vi "setting.vi"(7 "Level":i32, 10 "型号":string, 11 "型号表":string[](array[string])) -> (2 "型号out":string, 3 "型号表 out":string[](array[string]))   [LabVIEW 2025]
uses:
  global.vi
  <vilib>/Utility/config.llb/Read Key (String).vi
  <vilib>/Utility/config.llb/Write Key (String).vi
  <vilib>/Utility/config.llb/NI_LVConfig.lvlib
panel:
  in  "修改密码":bool caption="ChangePassword"
  in  "Tab":T1(tab)
  in  "CurrentType":enum16{"RMS均方根值", "AVG平均值"}(ring) caption="RMS/AVG Type"
  in  "最大电流":bool caption="Current Enabled"
  in  "平均电流":bool caption="RMS/AVG Enabled"
  in  "最大电流下限":dbl caption="Min Current" format="%#.2f"
  in  "平均电流下限":dbl caption="Min RMS/AVG" format="%#.2f"
  in  "平均电流上限":dbl caption="Max RMS/AVG" format="%#.2f"
  in  "最大电流上限":dbl caption="Max Current" format="%#.2f"
  in  "能量":bool caption="Power Enabled"
  in  "打钉时间":bool caption="Time Enabled"
  in  "能量下限":dbl caption="Min Power" format="%#.2f"
  in  "能量上限":dbl caption="Max Power" format="%#.2f"
  in  "时间下限":dbl caption="Min Time" format="%#.2f"
  in  "时间上限":dbl caption="Max Time" format="%#.2f"
  in  "检查数":dbl=20.0 caption="Check Stop Point"
  in  "PLCPort":string(combo) caption="PLC Port"
  in  "Language":string(combo)
  in  "最大补偿":dbl caption="Max Current  offset" format="%#.2f"
  in  "平均补偿":dbl caption="RMS/AVG Current offset" format="%#.2f"
  in  "能量补偿":dbl caption="Power offset" format="%#.2f"
  in  "时间补偿":dbl caption="Time offset" format="%#.2f"
  in  "单发打钉次数":u32=1 caption="Singe Times" min=1 max=20 step=1
  in  "连发打钉次数":u32=1 caption="Repeating Times" max=10 step=1
  in  "触发值":dbl caption="Trigger Level" format="%#.2f"
  in  "停止值":dbl caption="Stop Level" format="%#.2f"
  in  "倍数":dbl format="%#.2f"
  in  "HighVoltageAlarm":sgl=1.0 caption="High Voltage Alarm" min=1 max=50 step=0.5 format="%.2f"
  in  "LowVoltageAlarm":dbl=1.0 caption="Low Voltage Alarm" min=0.0 max=20.0 step=0.5 format="%.2f"
  in  "Modbus":string(combo)
  in  "另存为":bool caption="As Save"
  in  "退出":bool caption="Exit"
  in  "Save":bool
  # "A"
  # "A"
  # "A"
  # "A"
  # "ms"
  # "ms"
  # "A"
  # "A"
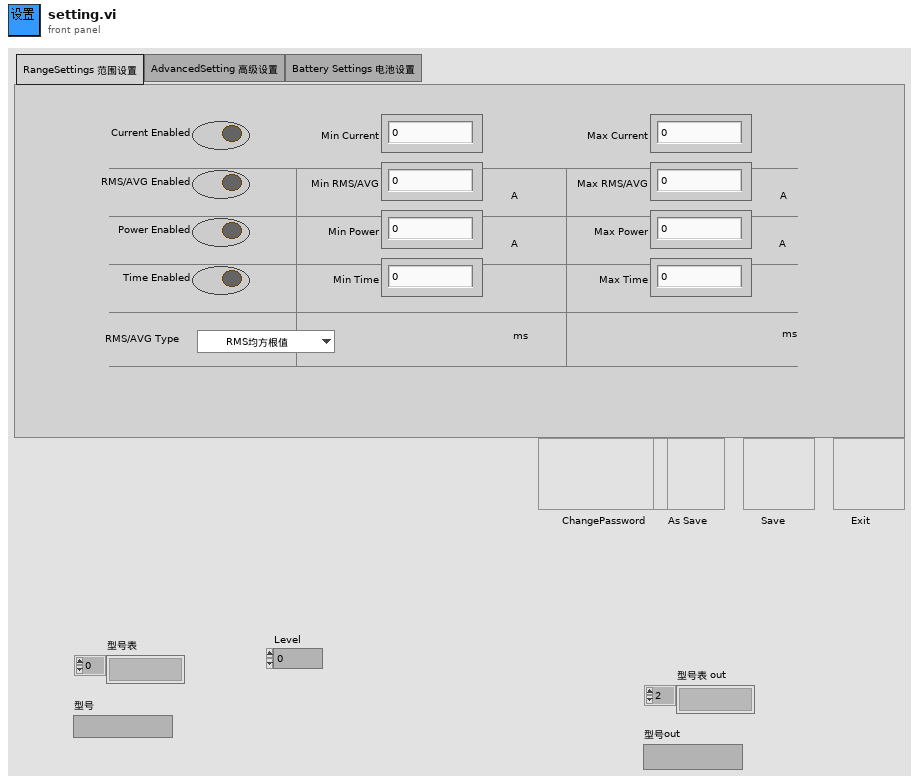
[diagram p1: front panel]
types:
  T1 = enum32{"RangeSettings 范围设置", "AdvancedSetting 高级设置", "Battery Settings 电池设置"}
  T2 = cluster{"Name":string, "Type":string, "DefVal":string}[]
  T3 = typedef "NI_LVConfig.lvlib/Config Data RefNum.ctl" = refnum<k1>
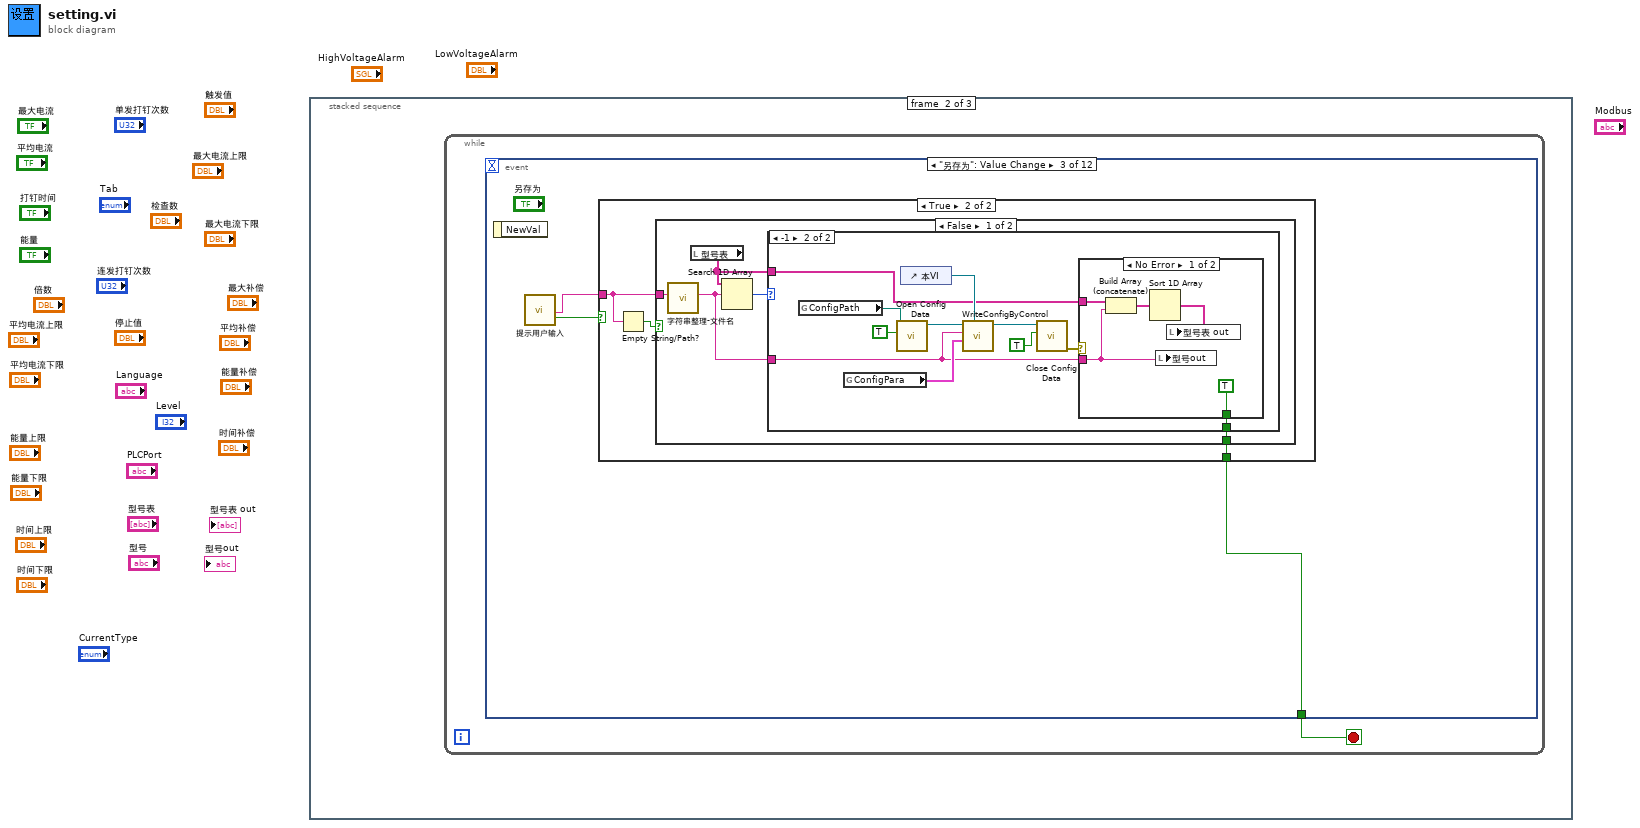
[diagram p0: block diagram]
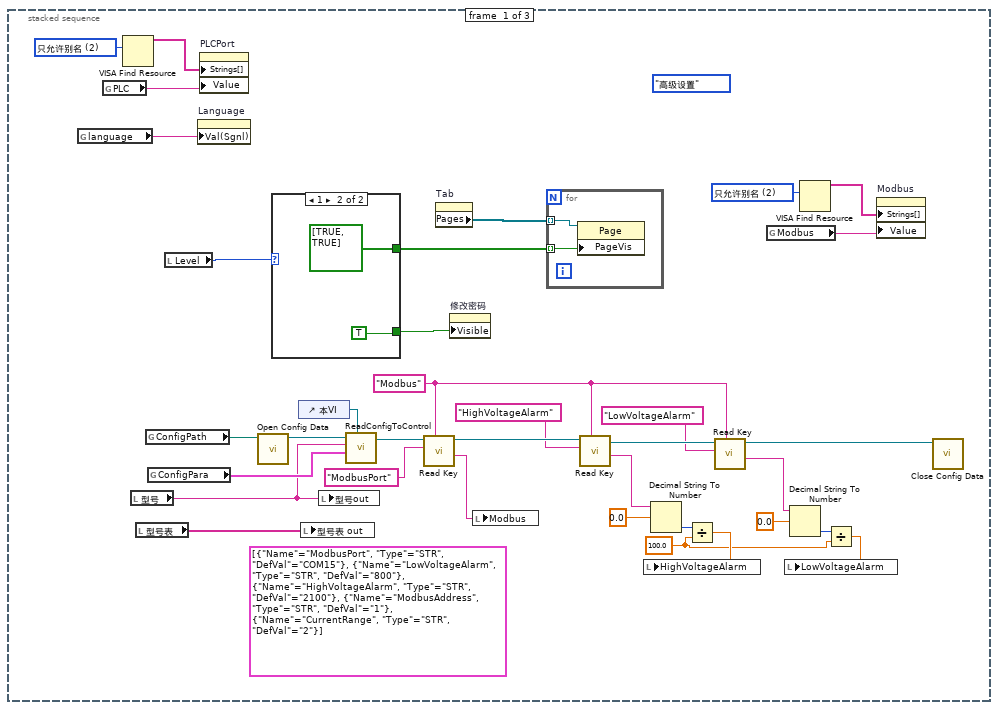
[diagram p2: hidden frame]
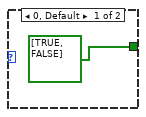
[diagram p3: hidden frame]
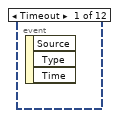
[diagram p4: hidden frame]
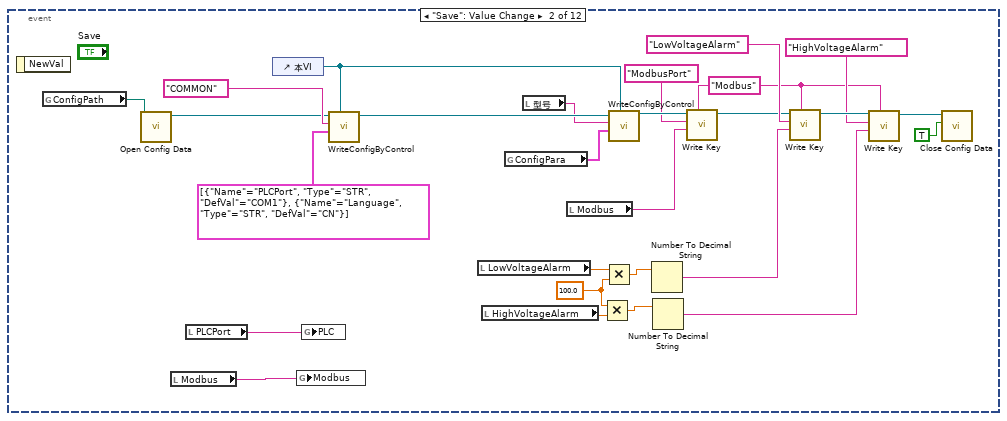
[diagram p5: hidden frame]
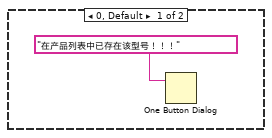
[diagram p7: hidden frame]
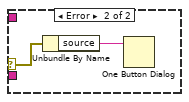
[diagram p8: hidden frame]
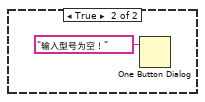
[diagram p9: hidden frame]
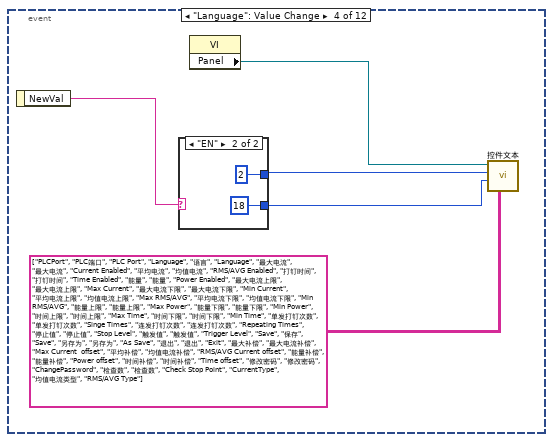
[diagram p10: hidden frame]
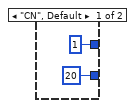
[diagram p11: hidden frame]
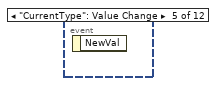
[diagram p12: hidden frame]
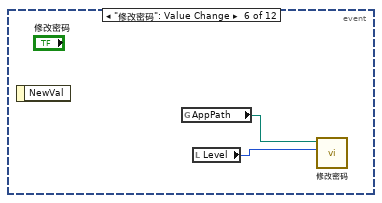
[diagram p13: hidden frame]
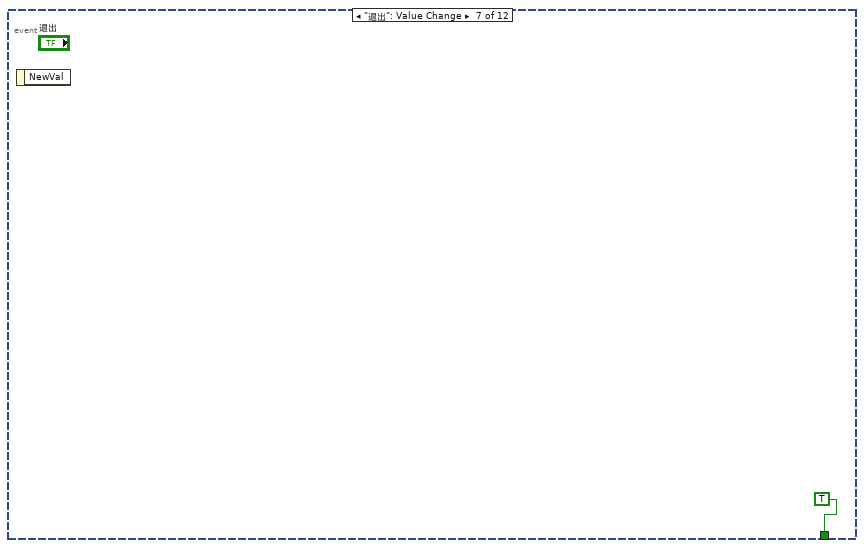
[diagram p14: hidden frame]
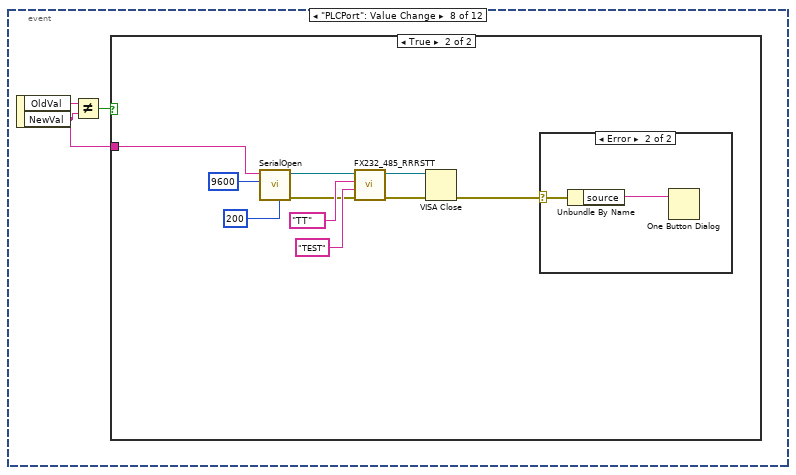
[diagram p15: hidden frame]
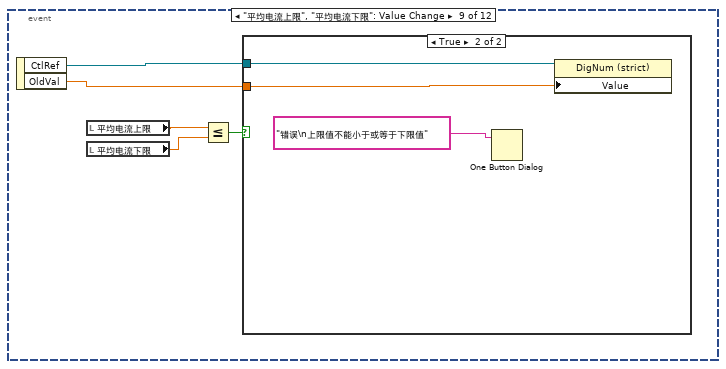
[diagram p18: hidden frame]
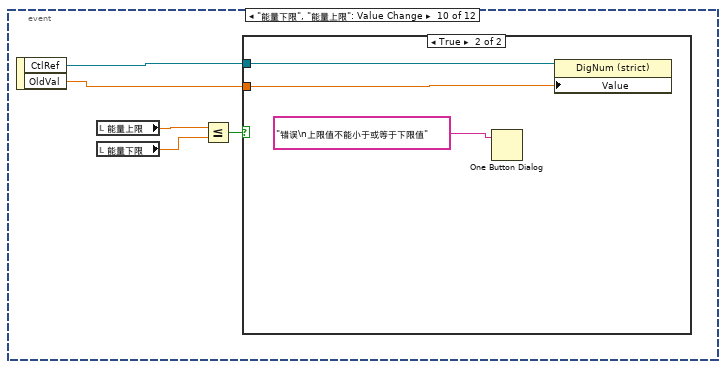
[diagram p20: hidden frame]
diagram:
  n1 = stacked-sequence {
    frame #0 {
      w1 = 100.0
      (unwired) T2 [{"Name"="ModbusPort", "Type"="STR", "DefVal"="COM15"}, {"Name"="LowVoltageAlarm", "Type"="STR", "DefVal"="800"}, {"Name"="HighVoltageAlarm", "Type"="STR", "DefVal"="2100"}, {"Name"="ModbusAddress", "Type"="STR", "DefVal"="1"}, {"Name"="CurrentRange", "Type"="STR", "DefVal"="2"}] ("ModbusConfig")
      w13 = "Modbus" ("section")
      w22 = u32 2 items=["仅允许规范名称"=0, "只允许别名"=2, "包含匹配别名"=3, "包含所有别名"=4] ("Search Mode")
      (unwired) enum32{"范围设置", "高级设置"}."高级设置" ("Tab")
      w35 = u32 2 items=["仅允许规范名称"=0, "只允许别名"=2, "包含匹配别名"=3, "包含所有别名"=4] ("Search Mode")
      n2 = global read "global.vi" "language"() -> (w33:string)
      n3 = global read "global.vi" "PLC"() -> (w32:string)
      n4 = VISA Find Resource(10:w35) -> (3:w34:string[])  [unwired: 2 in, 2 out]
      n5 = local read "型号"() -> (w28:string)
      n6 = local read "型号表"() -> (w27:string[])
      n7 = global read "global.vi" "ConfigPath"() -> (w31:path)
      n8 = global read "global.vi" "ConfigPara"() -> (w29:T2)
      n9 = local read "Level"() -> (w23:i32)
      n10 = property on="Language" class="CmbBox"("Val(Sgnl)"=w33) -> ()  [unwired: 2 in, 2 out]
      n11 = property on="PLCPort" class="CmbBox"("Strings[]"=w34, "Value"=w32) -> ()  [unwired: 2 in, 2 out]
      n12 = call <vilib>:"Open Config Data.vi"("configuration file path"=w31) -> ("refnum"=w30:T3)  [unwired: 8 in, 2 out]
      n13 = case shown="1" w23 {
        tunnel: [bool[] [TRUE, FALSE] bool[] [TRUE, TRUE]] -> w25
        tunnel: [_ TRUE] -> w24
        frame 0, Default {
        }
        frame 1 {
        }
      }
      n14 = control-ref of="本VI"() -> (w19:refnum<vi>)
      n15 = local write "型号表 out"(w27) -> ()
      n16 = local write "型号out"(w28) -> ()
      n17 = call "ReadConfigToControl.vi"("VI引用句柄"=w19, "ConfigInfo"=w29, "section"=w28, "refnum"=w30) -> ("refnum out"=w18:refnum<k1>)  [unwired: 6 in, 1 out]
      n18 = call-poly <vilib>:"Read Key.vi"("section"=w13, "key"="ModbusPort", "refnum"=w18) -> ("value"=w17:string, "refnum out"=w15:T3)  [unwired: 5 in, 2 out]
      n19 = property on="Tab" class="TabCtl (strict)"() -> ("Pages"=w26:refnum<vi>[])  [unwired: 2 in, 2 out]
      n20 = property on="修改密码" class="Bool"("Visible"=w24) -> ()  [unwired: 2 in, 2 out]
      n21 = local write "Modbus"(w17) -> ()
      n22 = for {
        tunnel: w26 -> [w40] mode=indexing
        tunnel: w25 -> [w39] mode=indexing
        n23 = property class="Page"(reference=w40, "PageVis"=w39) -> ()  [unwired: 1 in, 2 out]
      }
      n24 = call-poly <vilib>:"Read Key.vi"("section"=w13, "key"="HighVoltageAlarm", "refnum"=w15) -> ("value"=w9:string, "refnum out"=w12:T3)  [unwired: 5 in, 2 out]
      n25 = Decimal String To Number(string=w9, offset=0.0) -> (number=w7:i32)  [unwired: 1 in, 1 out]
      n26 = Divide(x=w7, y=w1) -> (x/y=w6:dbl)
      n27 = local write "HighVoltageAlarm"(w6) -> ()
      n28 = call-poly <vilib>:"Read Key.vi"("section"=w13, "key"="LowVoltageAlarm", "refnum"=w12) -> ("value"=w4:string, "refnum out"=w10:T3)  [unwired: 5 in, 2 out]
      n29 = global read "global.vi" "Modbus"() -> (w20:string)
      n30 = Decimal String To Number(string=w4, offset=0.0) -> (number=w5:i32)  [unwired: 1 in, 1 out]
      n31 = VISA Find Resource(10:w22) -> (3:w21:string[])  [unwired: 2 in, 2 out]
      n32 = Divide(x=w5, y=w1) -> (x/y=w2:dbl)
      n33 = local write "LowVoltageAlarm"(w2) -> ()
      n34 = property on="Modbus" class="CmbBox"("Strings[]"=w21, "Value"=w20) -> ()  [unwired: 2 in, 2 out]
      n35 = call <vilib>:"Close Config Data.vi"("refnum"=w10) -> ()  [unwired: 9 in, 2 out]
    }
    frame #1 {
      n36 = while {
        stop <- w41 stop-if-true
        n37 = event shown="[2] \"另存为\": Value Change" {
          selector: _ -> [_ _ _ _ _ _ _ _ _ _ _ _]
          dyn-events: _ -> [_ _ _ _ _ _ _ _ _ _ _ _]
          timeout: _ -> [_ _ _ _ _ _ _ _ _ _ _ _]
          tunnel: [_ _ w69 _ _ _ TRUE _ _ _ _ _] -> w41
          event Timeout {
            n38 = event-data() -> ()  [unwired: 1 in, 3 out]
          }
          event "Save": Value Change {
            w49 = 100.0 ("y")
            w46 = "Modbus" ("section")
            n39 = event-data() -> ()  [unwired: 1 in, 1 out]
            n40 = global read "global.vi" "ConfigPath"() -> (w68:path)
            n41 = call <vilib>:"Open Config Data.vi"("configuration file path"=w68) -> ("refnum"=w62:T3)  [unwired: 8 in, 2 out]
            n42 = local read "Modbus"() -> (w59:string)
            n43 = local read "PLCPort"() -> (w61:string)
            n44 = control-ref of="本VI"() -> (w58:refnum<vi>)
            n45 = global write "global.vi" "Modbus"(w59) -> ()
            n46 = global write "global.vi" "PLC"(w61) -> ()
            n47 = call "WriteConfigByControl.vi"("VI引用句柄"=w58, "ConfigInfo"=T2 [{"Name"="PLCPort", "Type"="STR", "DefVal"="COM1"}, {"Name"="Language", "Type"="STR", "DefVal"="CN"}], "section"="COMMON", "refnum"=w62) -> ("refnum out"=w64:refnum<k1>)  [unwired: 6 in, 1 out]
            n48 = local read "LowVoltageAlarm"() -> (w50:dbl)
            n49 = local read "HighVoltageAlarm"() -> (w48:sgl)
            n50 = global read "global.vi" "ConfigPara"() -> (w66:T2)
            n51 = local read "型号"() -> (w60:string)
            n52 = local read "Modbus"() -> (w42:string)
            n53 = Multiply(x=w49, y=w48) -> (x*y=w47:dbl)
            n54 = Multiply(x=w50, y=w49) -> (x*y=w51:dbl)
            n55 = call "WriteConfigByControl.vi"("VI引用句柄"=w58, "ConfigInfo"=w66, "section"=w60, "refnum"=w64) -> ("refnum out"=w45:refnum<k1>)  [unwired: 6 in, 1 out]
            n56 = Number To Decimal String(number=w51) -> (decimal integer string=w53:string)  [unwired: 1 in]
            n57 = Number To Decimal String(number=w47) -> (decimal integer string=w54:string)  [unwired: 1 in]
            n58 = call-poly <vilib>:"Write Key.vi"("section"=w46, "value"=w42, "key"="ModbusPort", "refnum"=w45) -> ("refnum out"=w44:T3)  [unwired: 5 in, 2 out]
            n59 = call-poly <vilib>:"Write Key.vi"("section"=w46, "value"=w53, "key"="LowVoltageAlarm", "refnum"=w44) -> ("refnum out"=w56:T3)  [unwired: 5 in, 2 out]
            n60 = call-poly <vilib>:"Write Key.vi"("section"=w46, "value"=w54, "key"="HighVoltageAlarm", "refnum"=w56) -> ("refnum out"=w52:T3)  [unwired: 5 in, 2 out]
            n61 = call <vilib>:"Close Config Data.vi"("write file if changed (T)"=TRUE, "refnum"=w52) -> ()  [unwired: 8 in, 2 out]
          }
          event "另存为": Value Change {
            n62 = event-data() -> ()  [unwired: 1 in, 1 out]
            n63 = call "提示用户输入"() -> ("产品型号"=w70:string, "确定"=w71:bool)  [unwired: 17 in, 1 out]
            n64 = case shown="True" w71 {
              tunnel: w70 -> [_ w73]
              tunnel: [_ w74] -> w69
              frame False {
              }
              frame True {
                n65 = Empty String/Path?(string/path=w73) -> (empty?=w72:bool)
                n66 = case shown="False" w72 {
                  tunnel: [w78 _] -> w74
                  tunnel: w73 -> [w76 _]
                  frame False {
                    n67 = call "字符串整理-文件名.vi"("输入字符串"=w76) -> ("结果字符串"=w77:string)  [unwired: 10 in]
                    n68 = local read "型号表"() -> (w75:string[])
                    n69 = Search 1D Array(1D array=w75, element=w77) -> (index of element=w79:i32)  [unwired: 1 in]
                    n70 = case shown="-1" w79 {
                      tunnel: w77 -> [_ w83]
                      tunnel: [_ w82] -> w78
                      tunnel: w75 -> [_ w81]
                      frame 0, Default {
                        n71 = One Button Dialog(message="在产品列表中已存在该型号！！！" ("消息")) -> ()  [unwired: 1 in, 1 out]
                      }
                      frame -1 {
                        n72 = global read "global.vi" "ConfigPath"() -> (w91:path)
                        n73 = global read "global.vi" "ConfigPara"() -> (w88:T2)
                        n74 = call <vilib>:"Open Config Data.vi"("create file if necessary (T)"=TRUE, "configuration file path"=w91) -> ("refnum"=w85:T3)  [unwired: 7 in, 2 out]
                        n75 = control-ref of="本VI"() -> (w86:refnum<vi>)
                        n76 = call "WriteConfigByControl.vi"("VI引用句柄"=w86, "ConfigInfo"=w88, "section"=w83, "refnum"=w85) -> ("refnum out"=w87:refnum<k1>)  [unwired: 6 in, 1 out]
                        n77 = call <vilib>:"Close Config Data.vi"("write file if changed (T)"=TRUE, "refnum"=w87) -> ("error out"=w84:errorcluster)  [unwired: 8 in, 1 out]
                        n78 = case shown="No Error" w84 {
                          selector: w84 -> [_ w98]
                          tunnel: w83 -> [w93 _]
                          tunnel: [TRUE _] -> w82
                          tunnel: w81 -> [w94 _]
                          frame No Error {
                            n79 = Build Array (concatenate)(w94, w93) -> (w92:string[])
                            n80 = Sort 1D Array(array=w92) -> (sorted array=w95:string[])
                            n81 = local write "型号out"(w93) -> ()
                            n82 = local write "型号表 out"(w95) -> ()
                          }
                          frame Error {
                            n83 = Unbundle By Name(w98) -> ("source"=w97:string)
                            n84 = One Button Dialog(message=w97) -> ()  [unwired: 1 in, 1 out]
                          }
                        }
                      }
                    }
                  }
                  frame True {
                    n85 = One Button Dialog(message="输入型号为空！" ("消息")) -> ()  [unwired: 1 in, 1 out]
                  }
                }
              }
            }
          }
          event "Language": Value Change {
            n86 = event-data() -> ("NewVal"=w104:string)  [unwired: 1 in]
            n87 = case shown="\"EN\"" w104 {
              tunnel: [1 ("禁用的索引 (列)") 2 ("禁用的索引 (列)")] -> w103
              tunnel: [u32 20 ("标题.字体:字号") u32 18 ("标题.字体:字号")] -> w102
              frame "CN", Default {
              }
              frame "EN" {
              }
            }
            n88 = property class="VI"() -> ("Panel"=w100:refnum<vi>)  [unwired: 2 in, 2 out]
            n89 = call "控件文本.vi"("数组"=string[][] [["PLCPort", "PLC端口", "PLC Port"], ["Language", "语言", "Language"], ["最大电流", "最大电流", "Current Enabled"], ["平均电流", "均值电流", "RMS/AVG Enabled"], ["打钉时间", "打钉时间", "Time Enabled"], ["能量", "能量", "Power Enabled"], ["最大电流上限", "最大电流上限", "Max Current"], ["最大电流下限", "最大电流下限", "Min Current"], ["平均电流上限", "均值电流上限", "Max RMS/AVG"], ["平均电流下限", "均值电流下限", "Min RMS/AVG"], ["能量上限", "能量上限", "Max Power"], ["能量下限", "能量下限", "Min Power"], ["时间上限", "时间上限", "Max Time"], ["时间下限", "时间下限", "Min Time"], ["单发打钉次数", "单发打钉次数", "Singe Times"], ["连发打钉次数", "连发打钉次数", "Repeating Times"], ["停止值", "停止值", "Stop Level"], ["触发值", "触发值", "Trigger Level"], ["Save", "保存", "Save"], ["另存为", "另存为", "As Save"], ["退出", "退出", "Exit"], ["最大补偿", "最大电流补偿", "Max Current  offset"], ["平均补偿", "均值电流补偿", "RMS/AVG Current offset"], ["能量补偿", "能量补偿", "Power offset"], ["时间补偿", "时间补偿", "Time offset"], ["修改密码", "修改密码", "ChangePassword"], ["检查数", "检查数", "Check Stop Point"], ["CurrentType", "均值电流类型", "RMS/AVG Type"]], "字号"=w102, "选择列"=w103, "引用"=w100) -> ()  [unwired: 8 in]
          }
          event "CurrentType": Value Change {
            n90 = event-data() -> ()  [unwired: 1 in, 1 out]
          }
          event "修改密码": Value Change {
            n91 = event-data() -> ()  [unwired: 1 in, 1 out]
            n92 = global read "global.vi" "AppPath"() -> (w109:path)
            n93 = local read "Level"() -> (w110:i32)
            n94 = call "修改密码.vi"("Level"=w110, "文件"=w109) -> ()  [unwired: 10 in]
          }
          event "退出": Value Change {
            n95 = event-data() -> ()  [unwired: 1 in, 1 out]
          }
          event "PLCPort": Value Change {
            n96 = event-data() -> ("OldVal"=w113:string, "NewVal"=w112:string)  [unwired: 1 in]
            n97 = Not Equal?(x=w113, y=w112) -> (x != y?=w114:bool)
            n98 = case shown="True" w114 {
              tunnel: w112 -> [_ w123]
              frame False {
              }
              frame True {
                n99 = call "SerialOpen.vi"("Timeout"=u32 200, "Baud Rate"=u32 9600, "Port"=w123) -> ("error out"=w117:errorcluster, "Port out"=w118:refnum<visa-resource-name>)  [unwired: 7 in]
                n100 = call "FX232_485_RRRSTT.vi"("error in (no error)"=w117, "值"="TEST", "命令"="TT", "Port"=w118) -> ("error out"=w115:errorcluster, "PortOut"=w116:refnum<visa-resource-name>)  [unwired: 4 in, 2 out]
                n101 = VISA Close(VISA resource name=w116, error in (no error)=w115) -> (error out=w124:errorcluster)
                n102 = case shown="Error" w124 {
                  selector: w124 -> [_ w126]
                  frame No Error {
                  }
                  frame Error {
                    n103 = Unbundle By Name(w126) -> ("source"=w125:string)
                    n104 = One Button Dialog(message=w125) -> ()  [unwired: 1 in, 1 out]
                  }
                }
              }
            }
          }
          event "平均电流上限", "平均电流下限": Value Change {
            n105 = event-data() -> ("CtlRef"=w130:refnum<vi>, "OldVal"=w129:dbl)  [unwired: 1 in]
            n106 = local read "平均电流上限"() -> (w128:dbl)
            n107 = local read "平均电流下限"() -> (w127:dbl)
            n108 = Less Or Equal?(x=w128, y=w127) -> (x <= y?=w131:bool)
            n109 = case shown="True" w131 {
              tunnel: w129 -> [_ w134]
              tunnel: w130 -> [_ w133]
              frame False {
              }
              frame True {
                n110 = One Button Dialog(message="错误\n上限值不能小于或等于下限值" ("Titre")) -> ()  [unwired: 1 in, 1 out]
                n111 = property class="DigNum (strict)"(reference=w133, "Value"=w134) -> ()  [unwired: 1 in, 2 out]
              }
            }
          }
          event "能量下限", "能量上限": Value Change {
            n112 = event-data() -> ("CtlRef"=w138:refnum<vi>, "OldVal"=w137:dbl)  [unwired: 1 in]
            n113 = local read "能量上限"() -> (w136:dbl)
            n114 = local read "能量下限"() -> (w135:dbl)
            n115 = Less Or Equal?(x=w136, y=w135) -> (x <= y?=w139:bool)
            n116 = case shown="True" w139 {
              tunnel: w137 -> [_ w142]
              tunnel: w138 -> [_ w141]
              frame False {
              }
              frame True {
                n117 = One Button Dialog(message="错误\n上限值不能小于或等于下限值" ("Titre")) -> ()  [unwired: 1 in, 1 out]
                n118 = property class="DigNum (strict)"(reference=w141, "Value"=w142) -> ()  [unwired: 1 in, 2 out]
              }
            }
          }
          event "时间上限", "时间下限": Value Change {
            n119 = event-data() -> ("CtlRef"=w146:refnum<vi>, "OldVal"=w145:dbl)  [unwired: 1 in]
            n120 = local read "时间上限"() -> (w144:dbl)
            n121 = local read "时间下限"() -> (w143:dbl)
            n122 = Less Or Equal?(x=w144, y=w143) -> (x <= y?=w147:bool)
            n123 = case shown="True" w147 {
              tunnel: w145 -> [_ w150]
              tunnel: w146 -> [_ w149]
              frame False {
              }
              frame True {
                n124 = One Button Dialog(message="错误\n上限值不能小于或等于下限值" ("Titre")) -> ()  [unwired: 1 in, 1 out]
                n125 = property class="DigNum (strict)"(reference=w149, "Value"=w150) -> ()  [unwired: 1 in, 2 out]
              }
            }
          }
          event "最大电流下限", "最大电流上限": Value Change {
            n126 = event-data() -> ("CtlRef"=w153:refnum<vi>, "OldVal"=w154:dbl)  [unwired: 1 in]
            n127 = local read "最大电流下限"() -> (w151:dbl)
            n128 = local read "最大电流上限"() -> (w152:dbl)
            n129 = Less Or Equal?(x=w152, y=w151) -> (x <= y?=w155:bool)
            n130 = case shown="True" w155 {
              tunnel: w154 -> [_ w158]
              tunnel: w153 -> [_ w157]
              frame False {
              }
              frame True {
                n131 = One Button Dialog(message="错误\n上限值不能小于或等于下限值" ("Titre")) -> ()  [unwired: 1 in, 1 out]
                n132 = property class="DigNum (strict)"(reference=w157, "Value"=w158) -> ()  [unwired: 1 in, 2 out]
              }
            }
          }
        }
      }
    }
    frame #2 {
      n133 = flat-sequence {
        frame #0 {
          n134 = global read "global.vi" "language"() -> (w160:string)
          n135 = local read "Language"() -> (w159:string)
          n136 = Not Equal?(x=w160, y=w159) -> ()  [unwired: 1 out]
          n137 = global write "global.vi" "language"(w159) -> ()
        }
        frame #1 {
          n138 = invoke class="VI" method="FP.Close"() -> ()  [unwired: 3 in, 3 out]
        }
      }
    }
  }
